vi "PicoScope2000UnitInfo.vi"(4 "handle in":i16=1, 5 "error in (no error)":errorcluster) -> (0 "Unit Info":T1, 1 "handle out":i16=1, 2 "error out":errorcluster)   [LabVIEW 2010]
uses:
  ps2000.dll
panel:
  out "status":i16
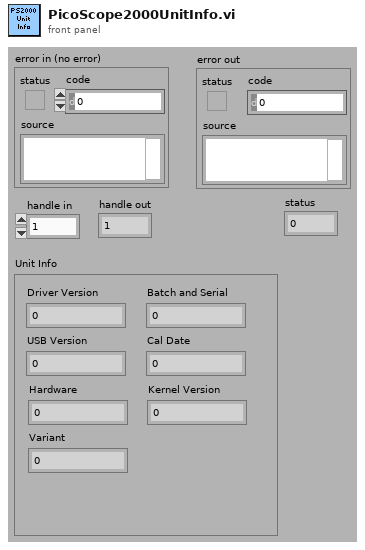
[diagram p1: front panel]
types:
  T1 = cluster{"Driver Version":string, "USB Version":string, "Hardware":string, "Variant":string, "Batch and Serial":string, "Cal Date":string, "Kernel Version":string}
  T2 = cluster{"[0]":string, "[1]":string, "[2]":string, "[3]":string, "[4]":string, "[5]":string, "[6]":string}
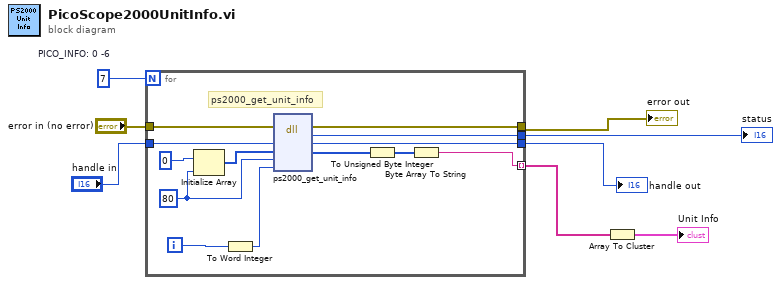
[diagram p0: block diagram]
diagram:
  w7 = 7  # PICO_INFO: 0 -6
  n1 = for {
    N: w7 -> [_]
    tunnel: "handle in" -> [w21]
    tunnel: "error in (no error)" -> [w20]
    tunnel: [w19] -> w5
    tunnel: [w18] -> w4
    tunnel: [w17] -> w1
    tunnel: [w9] -> w2 mode=indexing
    i -> [w16]
    w12 = i16 80 ("stringLength")
    # "ps2000_get_unit_info"
    n2 = Initialize Array(i8 0 ("element"), w12) -> (w13:i8[])
    n3 = To Word Integer(number=w16) -> (16bit integer=w15:i16)
    n4 = dll-call lib="PS2000.dll" fn="ps2000_get_unit_info"(error in=w20, "handle"=w21, "unitInfo"=w13, "stringLength"=w12, "line"=w15) -> (error out=w18:errorcluster, "status"=w17:i16, "handle"=w19:i16, "unitInfo"=w10:i8[])  [unwired: 4 in, 1 out]
    n5 = To Unsigned Byte Integer(number=w10) -> (unsigned 8bit integer=w11:u8[])
    n6 = Byte Array To String(unsigned byte array=w11) -> (string=w9:string)
  }
  "error out" <- w4
  "handle out" <- w5
  "status" <- w1
  n7 = Array To Cluster(array=w2) -> (cluster=→"Unit Info":T2)
